vi "ControllerUI_New_Final.vi"() -> ()   [LabVIEW 2026]
uses:
  <vilib>/Utility/error.llb/Trim Whitespace One-Sided.vi
  <userlib>/_OpenG.lib/file/file.llb/openg_file.lvlib
panel:
  in  "Tab Control":T1(tab)
  out "background 2":picture
  in  "5-Day Rainstorm-to-Flood":bool
  out "script Status":string
  in  "voltage 1":dbl
  in  "DESD4 SOC":dbl(slide) step=1.0 scale=0.0..100.0 scale format="%#.6g"
  in  "DESD3 SOC":dbl(slide) step=1.0 scale=0.0..100.0 scale format="%#.6g"
  in  "DESD2 SOC":dbl(slide) step=1.0 scale=0.0..100.0 scale format="%#.6g"
  in  "wind speed":dbl(knob) caption="Wind Speed (m/s)" min=0.0 max=30.0 step=0.5 scale=0.0..255.0
  in  "stop":bool
  in  "Send UDP Command":bool caption="IO Building Send"
  out "Device Badge":string
  out "Selected Summary":string
  out "Device Description":string
  out "Device Name":string
  in  "DESD1 SOC":dbl(slide) step=1.0 scale=0.0..100.0 scale format="%#.6g"
  in  "BTN_DESD_4":bool
  in  "BTN_PV_1":bool
  in  "BTN_DESD_2":bool
  in  "BTN_Gen_1":bool
  in  "BTN_DESD_1":bool
  in  "BTN_Gen_2":bool
  in  "BTN_DESD_3":bool
  in  "BTN_PV_2":bool
  in  "BTN_Load_2":bool
  in  "BTN_Load_4":bool
  in  "BTN_Grid_1":bool
  in  "BTN_Load_3":bool
  in  "BTN_Wind_Turbine":bool
  out "background":picture
  in  "IO 1":bool
  in  "IO 2":bool
  in  "IO 3":bool
  in  "IO 4":bool
  in  "IO 6":bool
  in  "IO 7":bool
  in  "IO 8":bool
  in  "IO 5":bool
  in  "IO 9":bool
  in  "IO 10":bool
  in  "IO 11":bool
  in  "IO 12":bool
  in  "IO 13":bool
  in  "IO 14":bool
  in  "IO 15":bool
  in  "IO 16":bool
  in  "voltage 2":dbl
  in  "voltage 3":dbl
  in  "voltage 4":dbl
  # "LabVIEW-Based Physical Sandbox Intelligent Control System"
  # "LabVIEW-Based Physical Sandbox Intelligent Control System"
  # "Node Information"
  # "Control Panel"
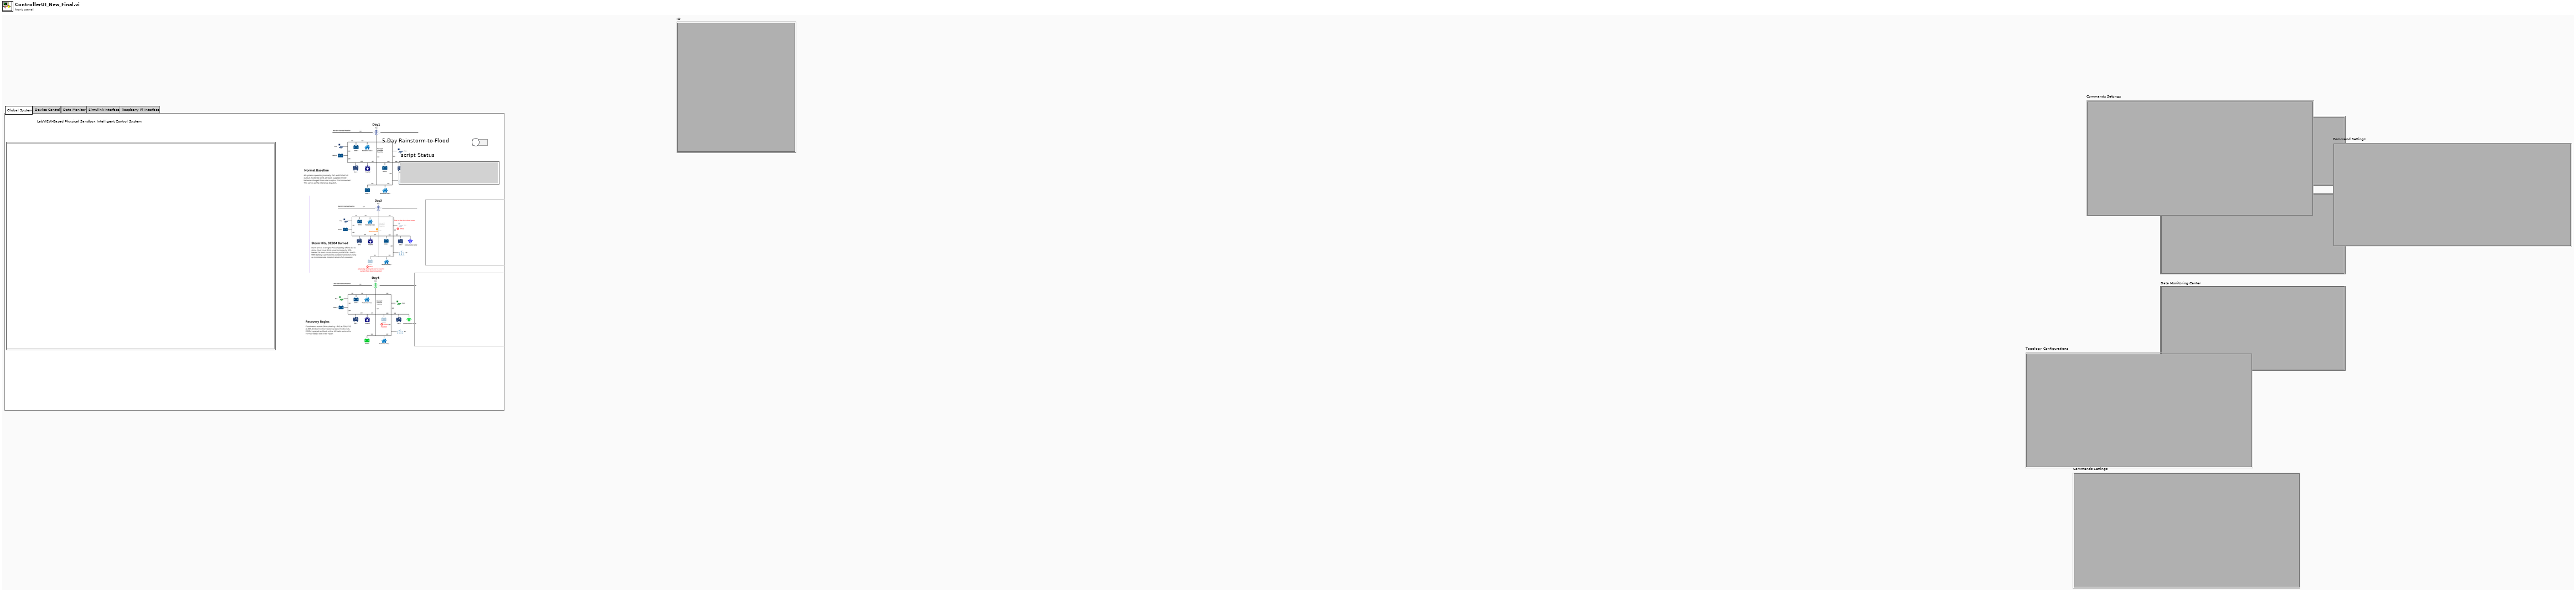
[diagram p1: front panel]
types:
  T1 = enum32{"Global System", "Device Control", "Data Monitor", "Simulink Interface", "Raspberry Pi Interface"}
  T2 = typedef "imagedata.ctl" = cluster{"image type":i32, "image depth":i32, "image":u8[], "mask":u8[], "colors":u32[], "Rectangle":cluster{"left":i16, "top":i16, "right":i16, "bottom":i16}}
  T3 = cluster{string, "wind speed":dbl, i32, i32, i32, i32}
  T4 = cluster{string, " DESD4 SOC":dbl, dbl, dbl, i32, i32}
  T5 = cluster{string, " DESD3 SOC":dbl, dbl, dbl, i32, i32}
  T6 = cluster{string, " DESD2 SOC":dbl, dbl, dbl, i32, i32}
  T7 = cluster{string, " DESD1 SOC":dbl, dbl, dbl, i32, i32}
  T8 = cluster{string, " DESD4 SOC":dbl, dbl, dbl, i32, i32}[]
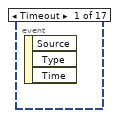
[diagram p2: hidden frame]
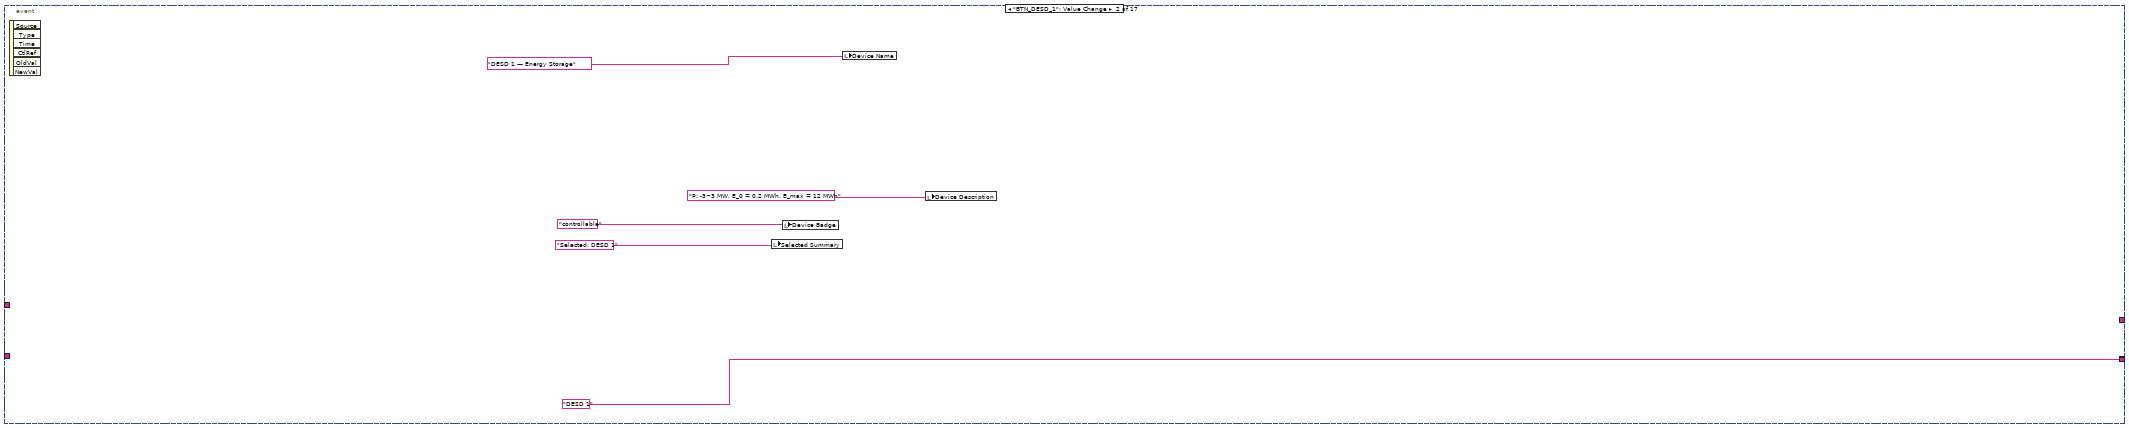
[diagram p3: hidden frame]
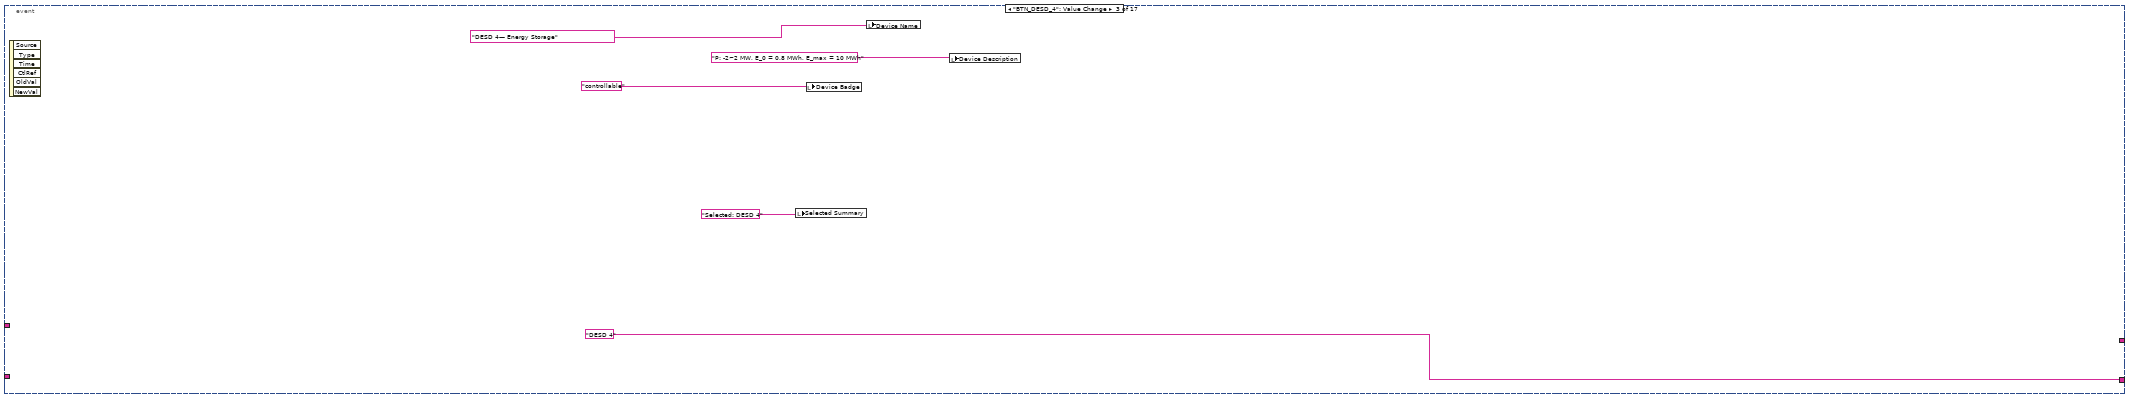
[diagram p4: hidden frame]
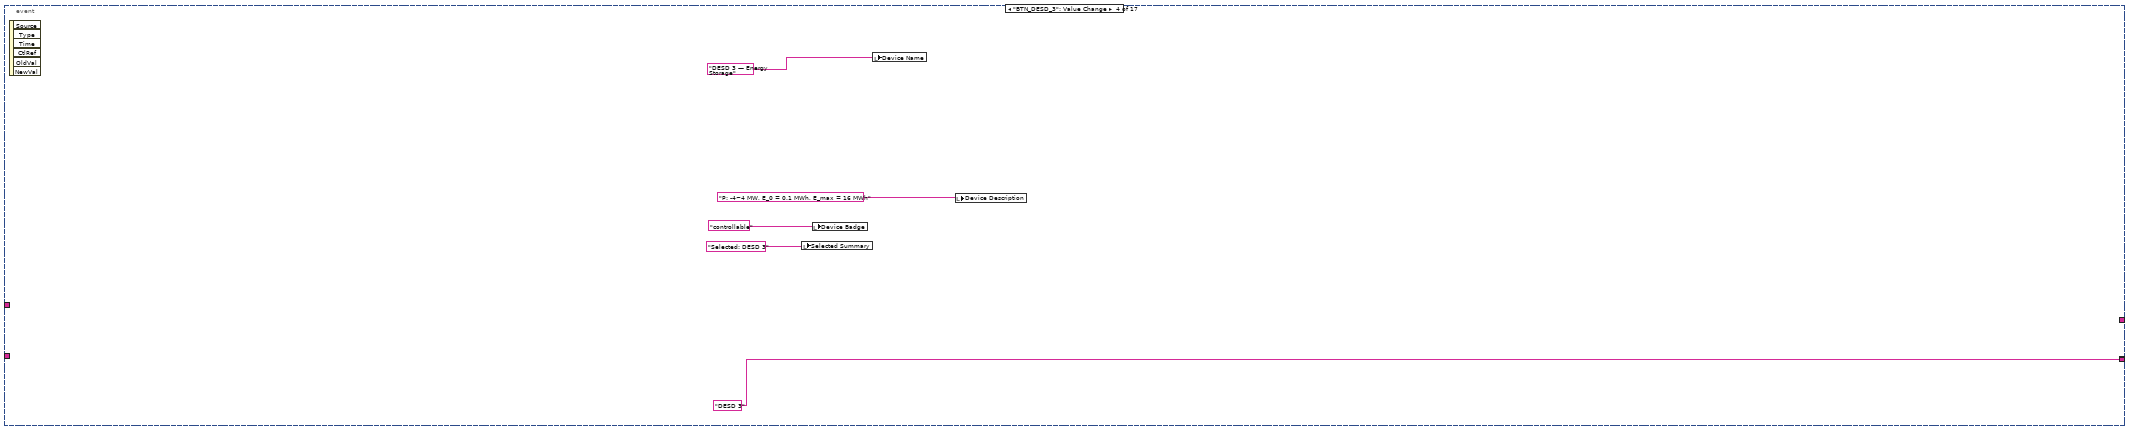
[diagram p5: hidden frame]
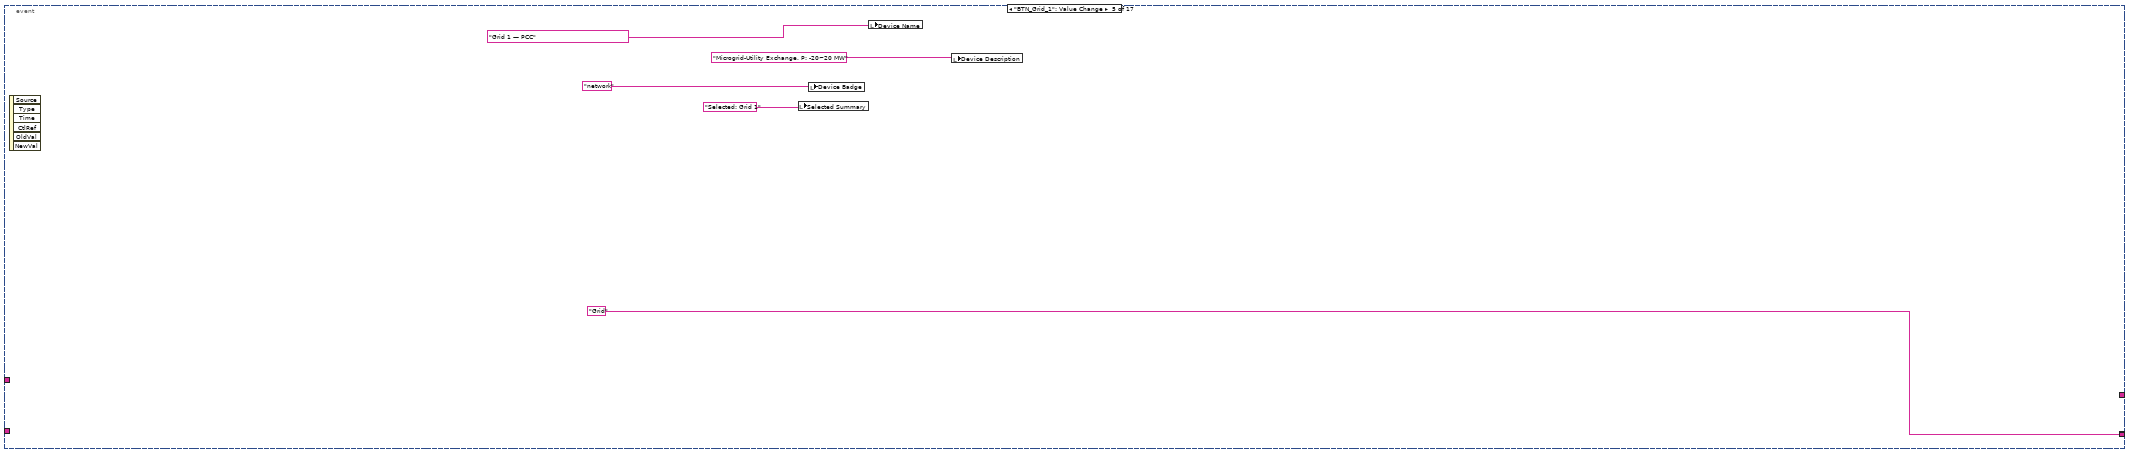
[diagram p6: hidden frame]
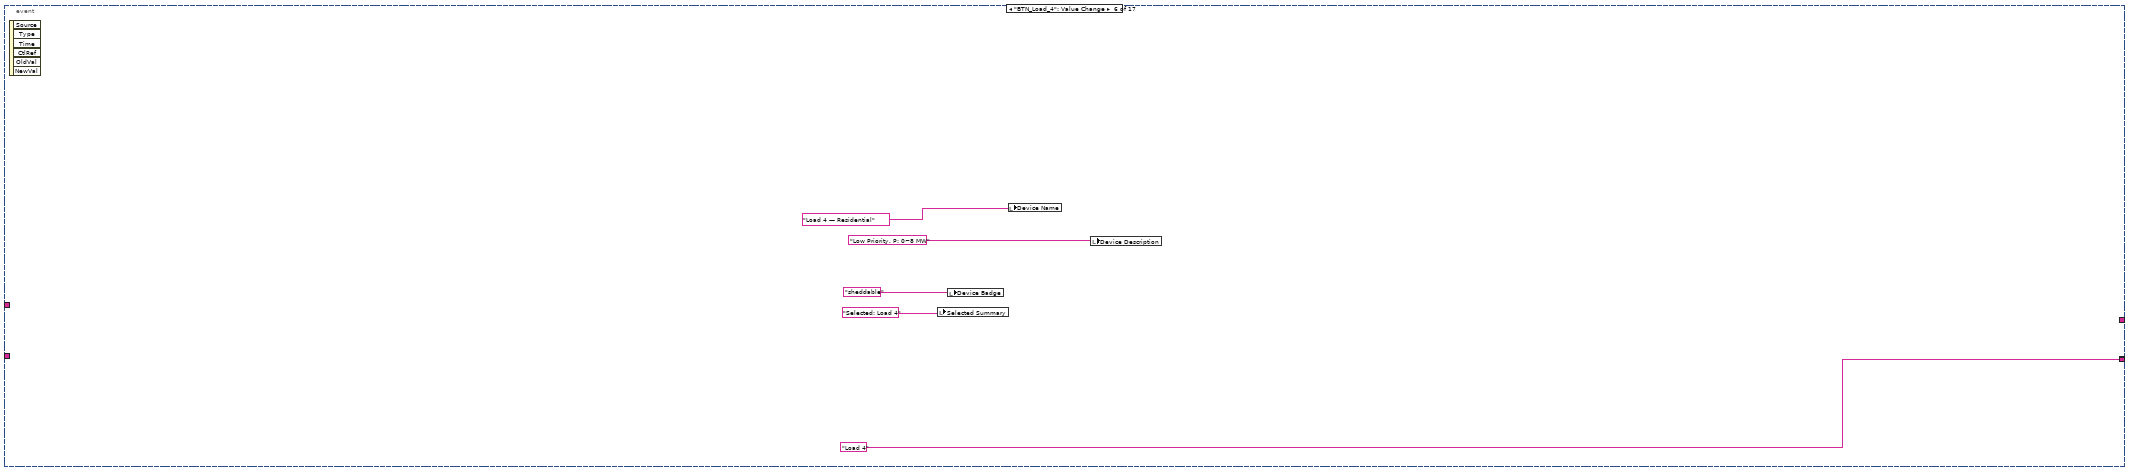
[diagram p7: hidden frame]
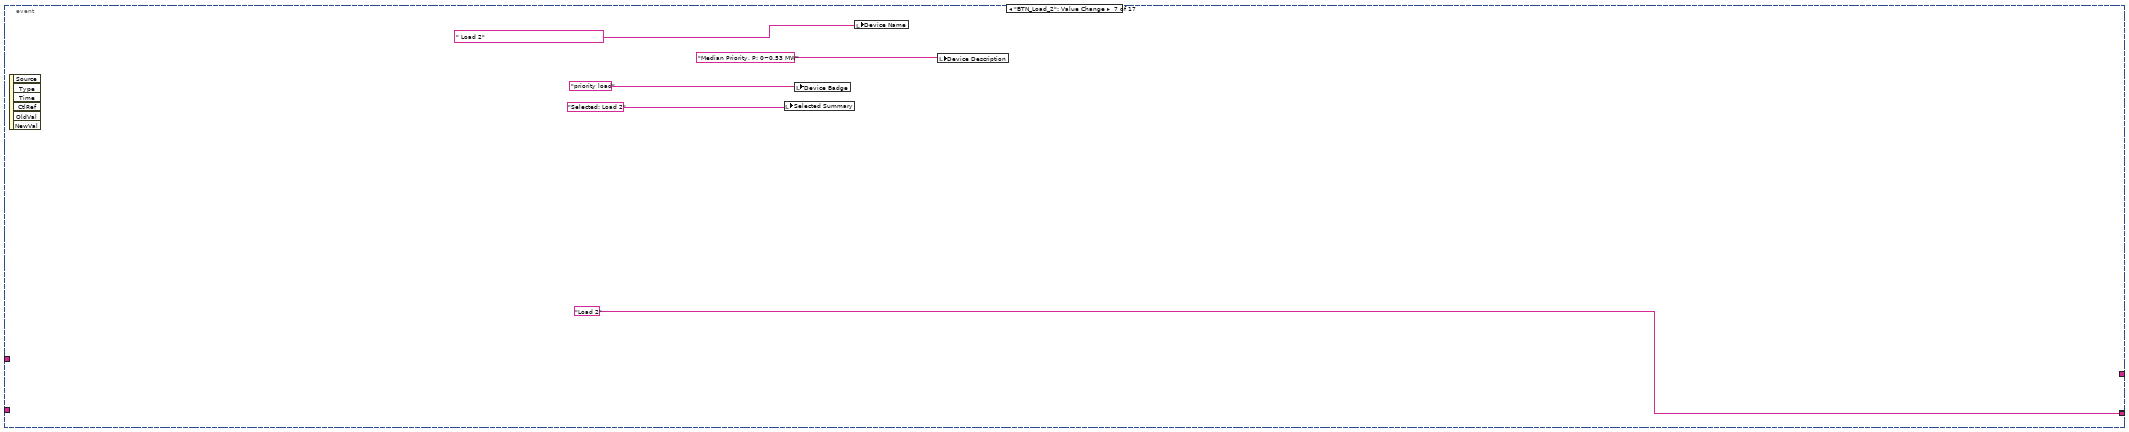
[diagram p8: hidden frame]
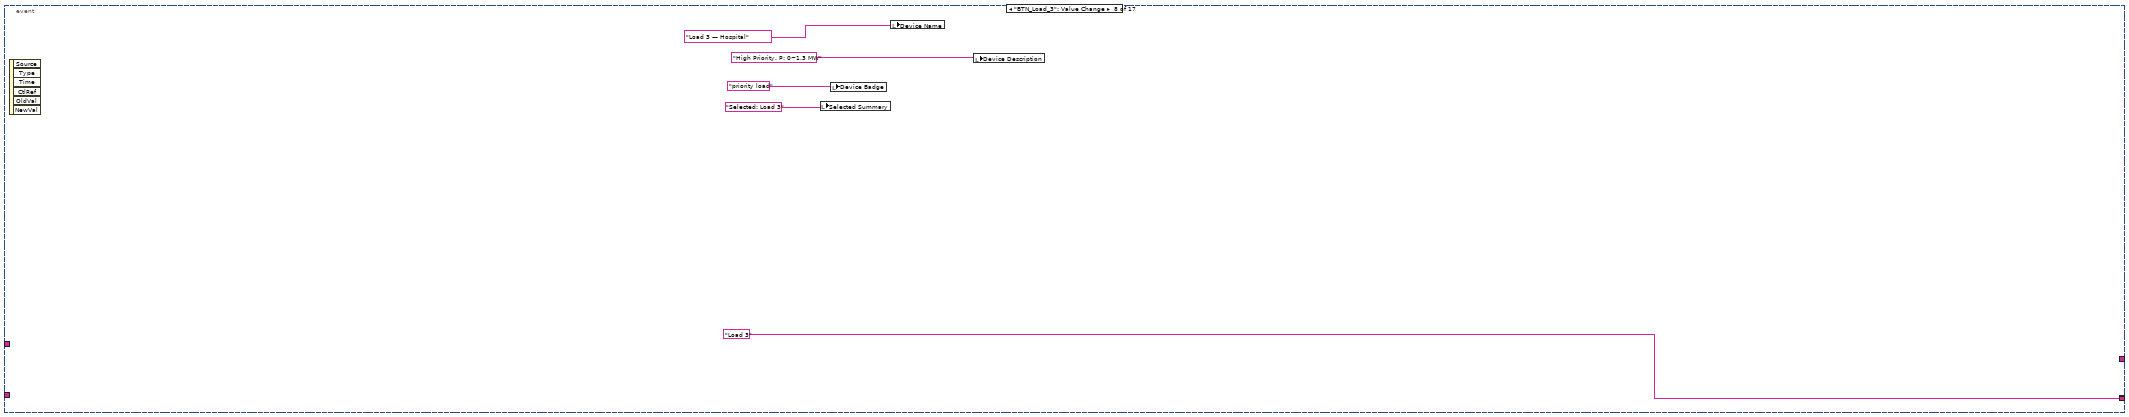
[diagram p9: hidden frame]
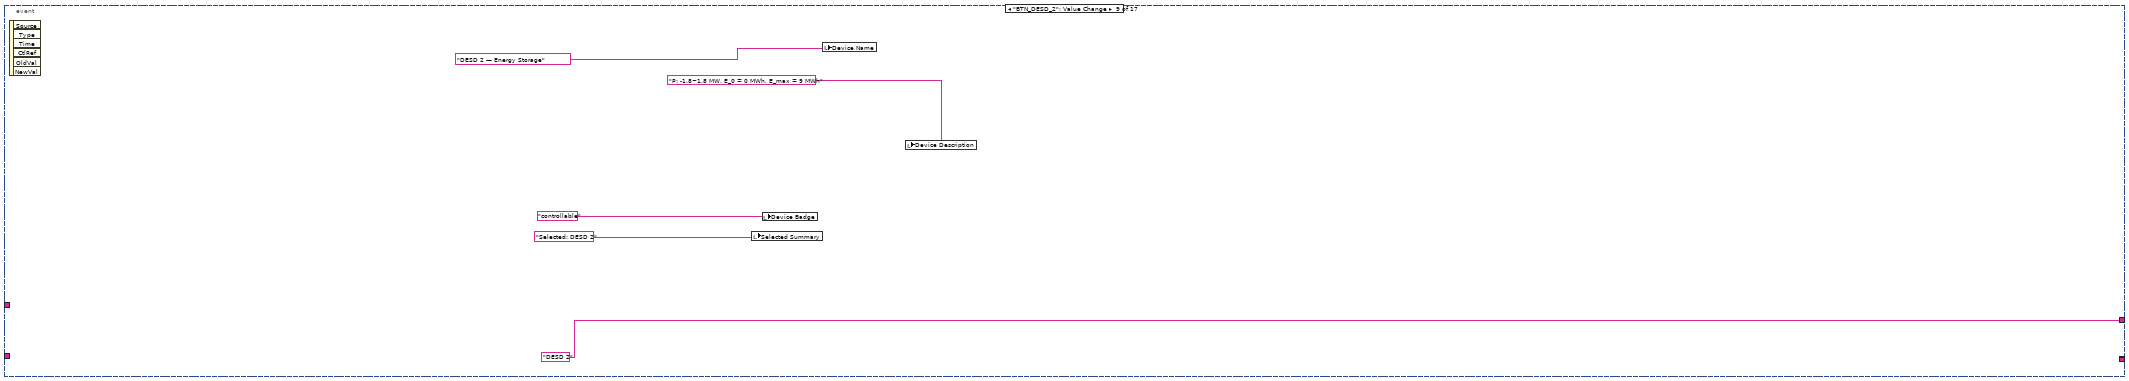
[diagram p10: hidden frame]
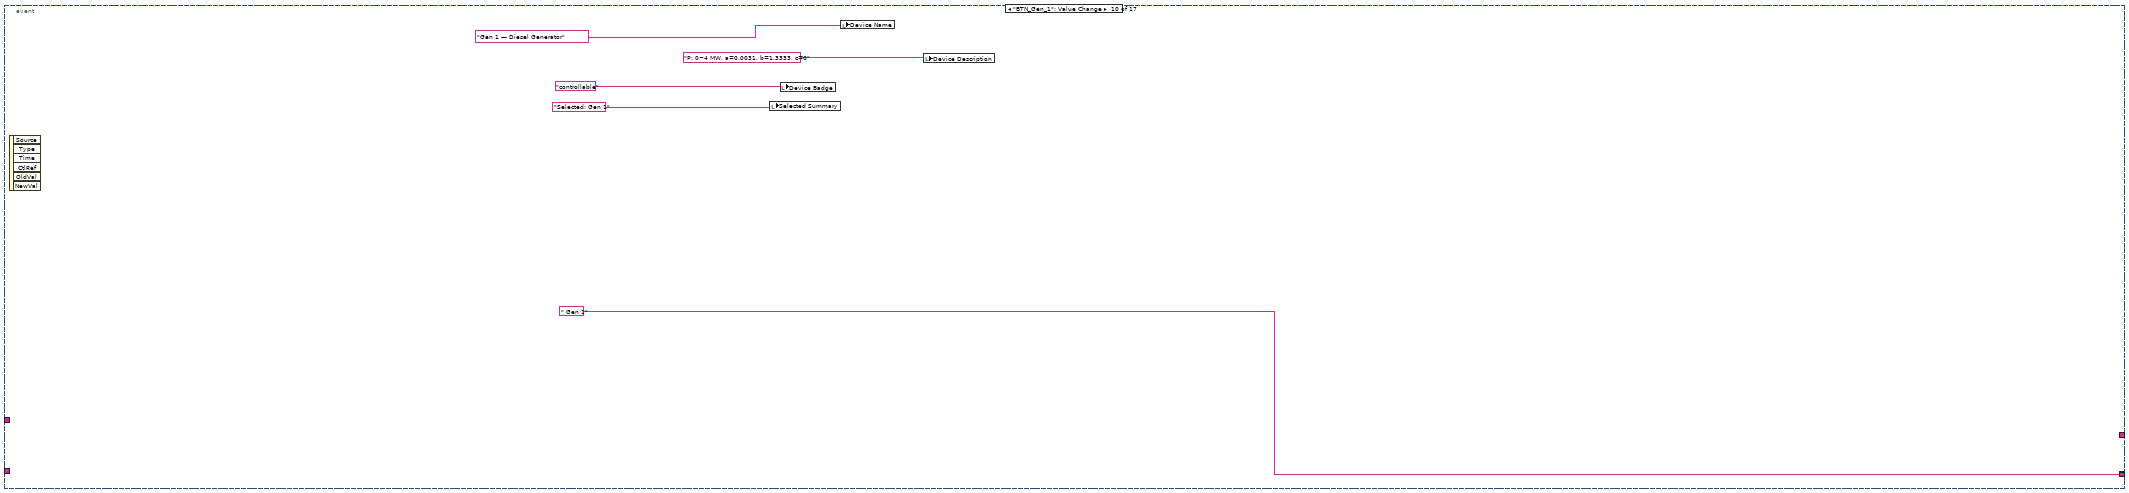
[diagram p11: hidden frame]
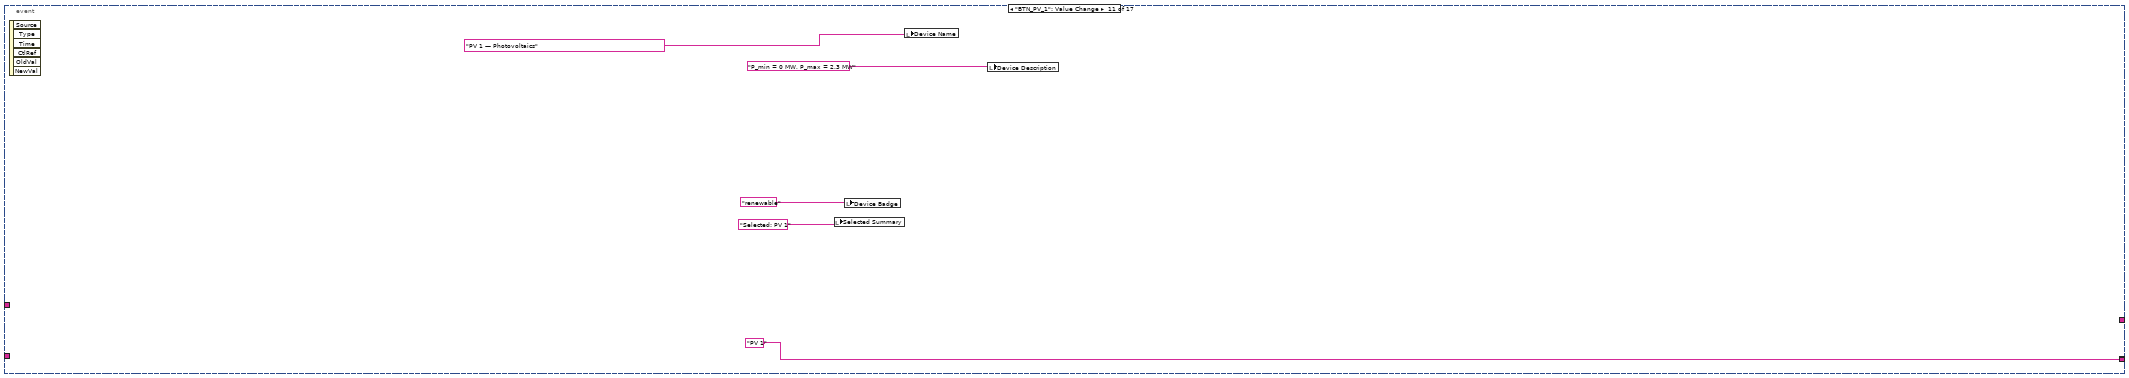
[diagram p12: hidden frame]
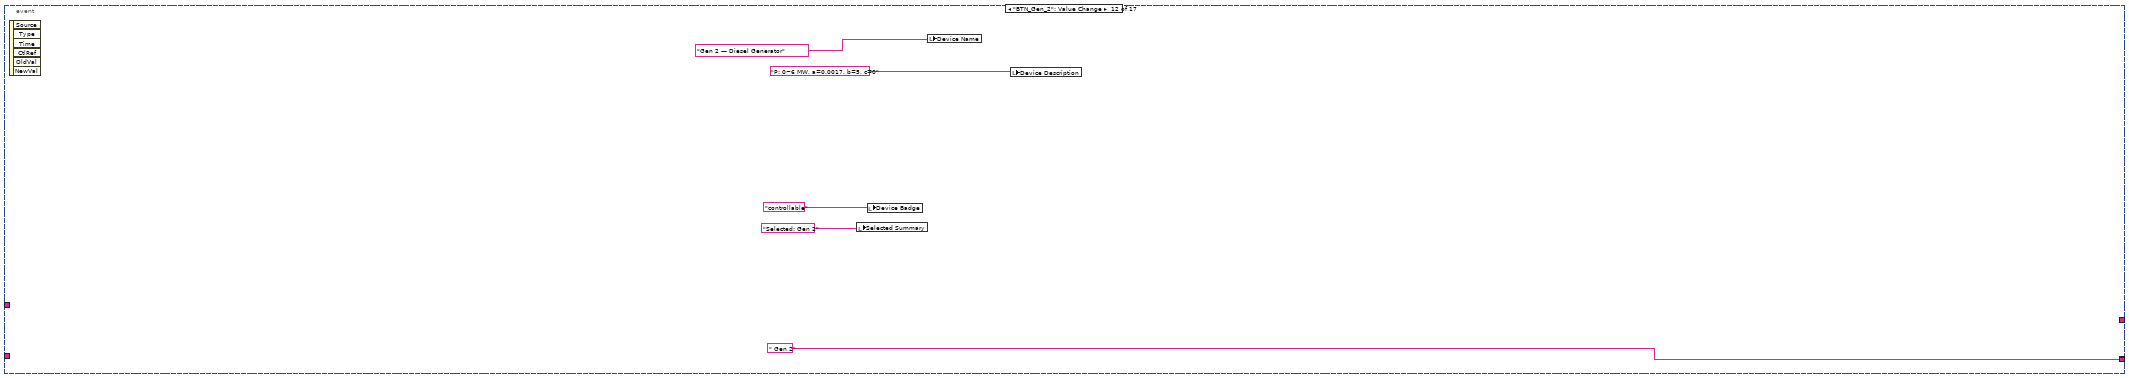
[diagram p13: hidden frame]
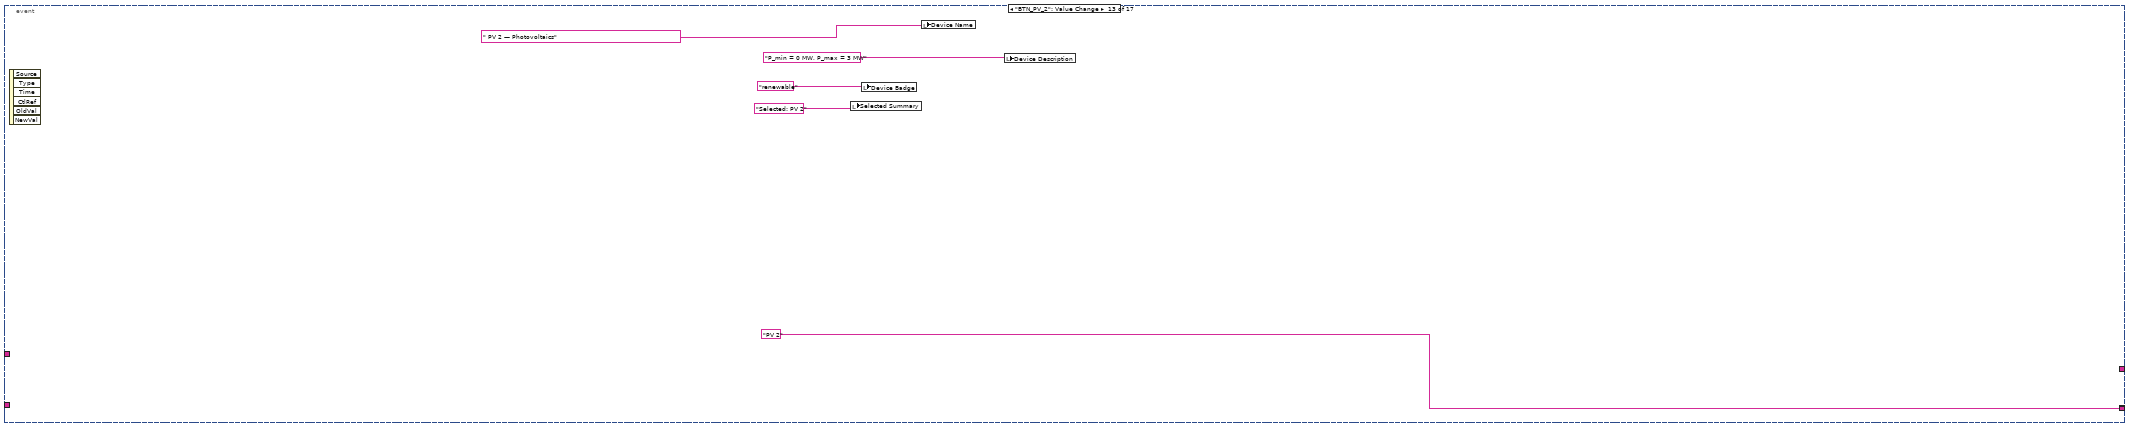
[diagram p14: hidden frame]
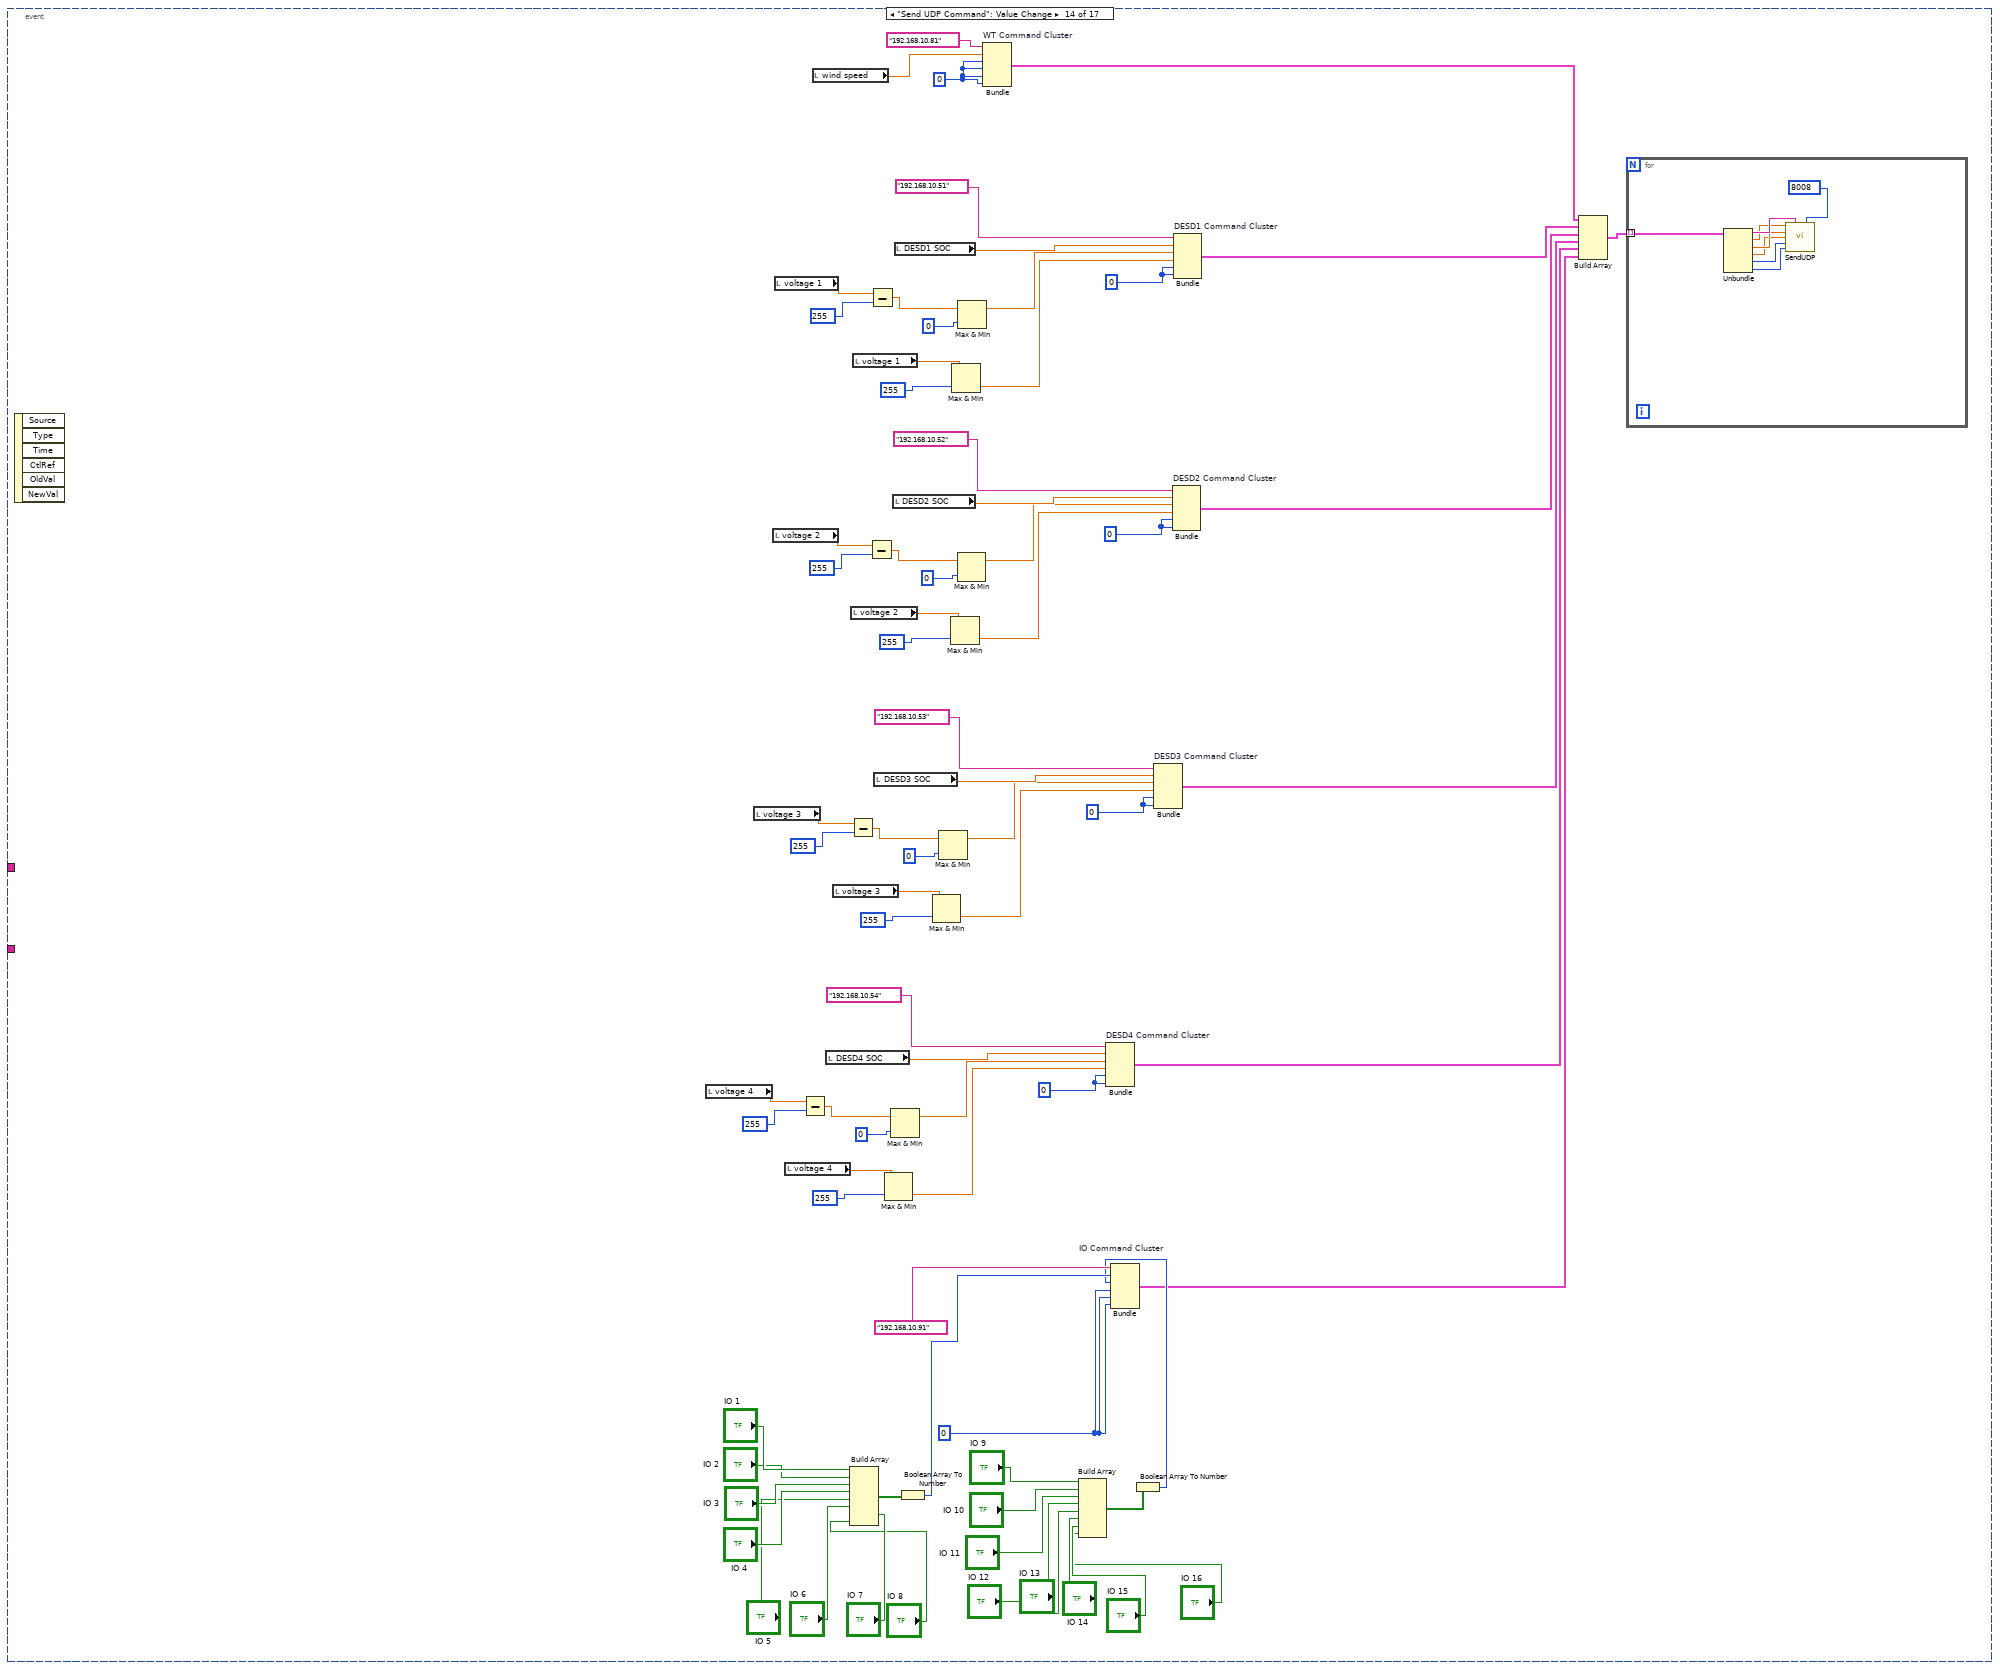
[diagram p15: hidden frame]
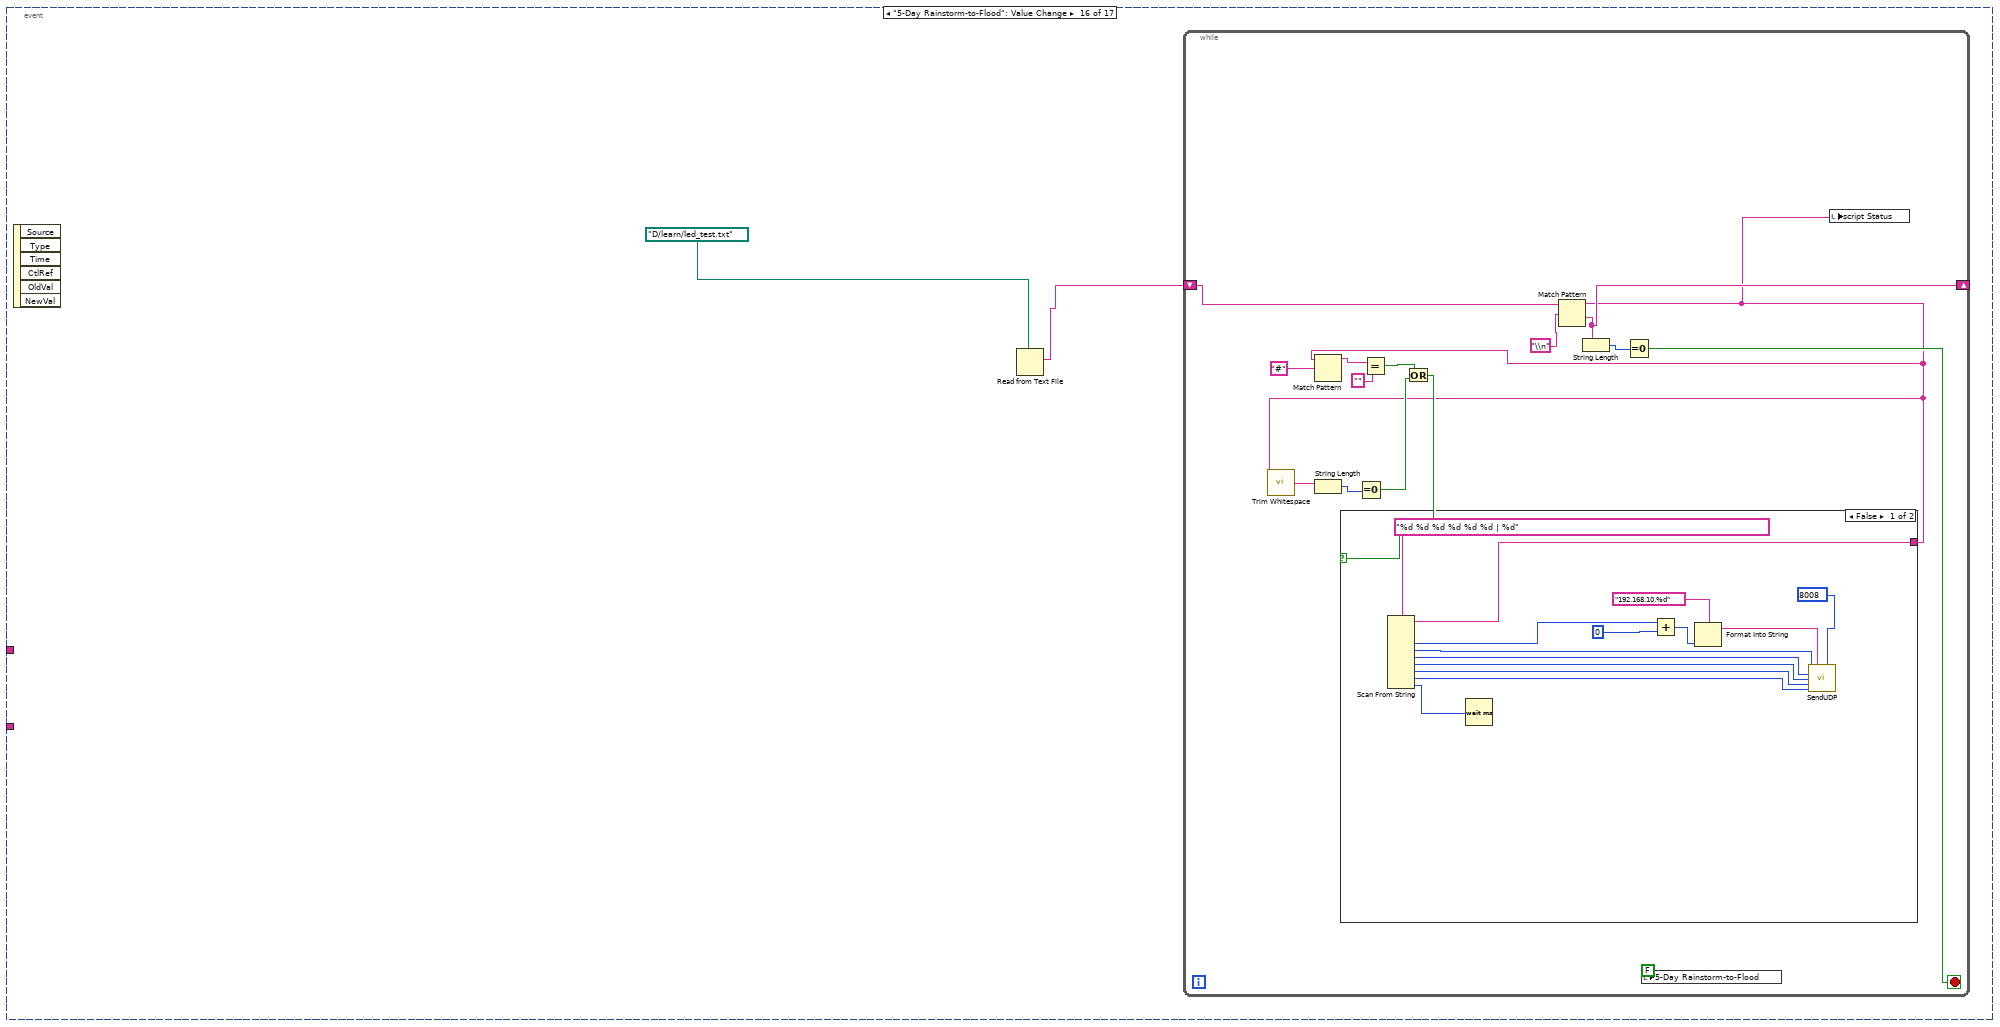
[diagram p16: hidden frame]
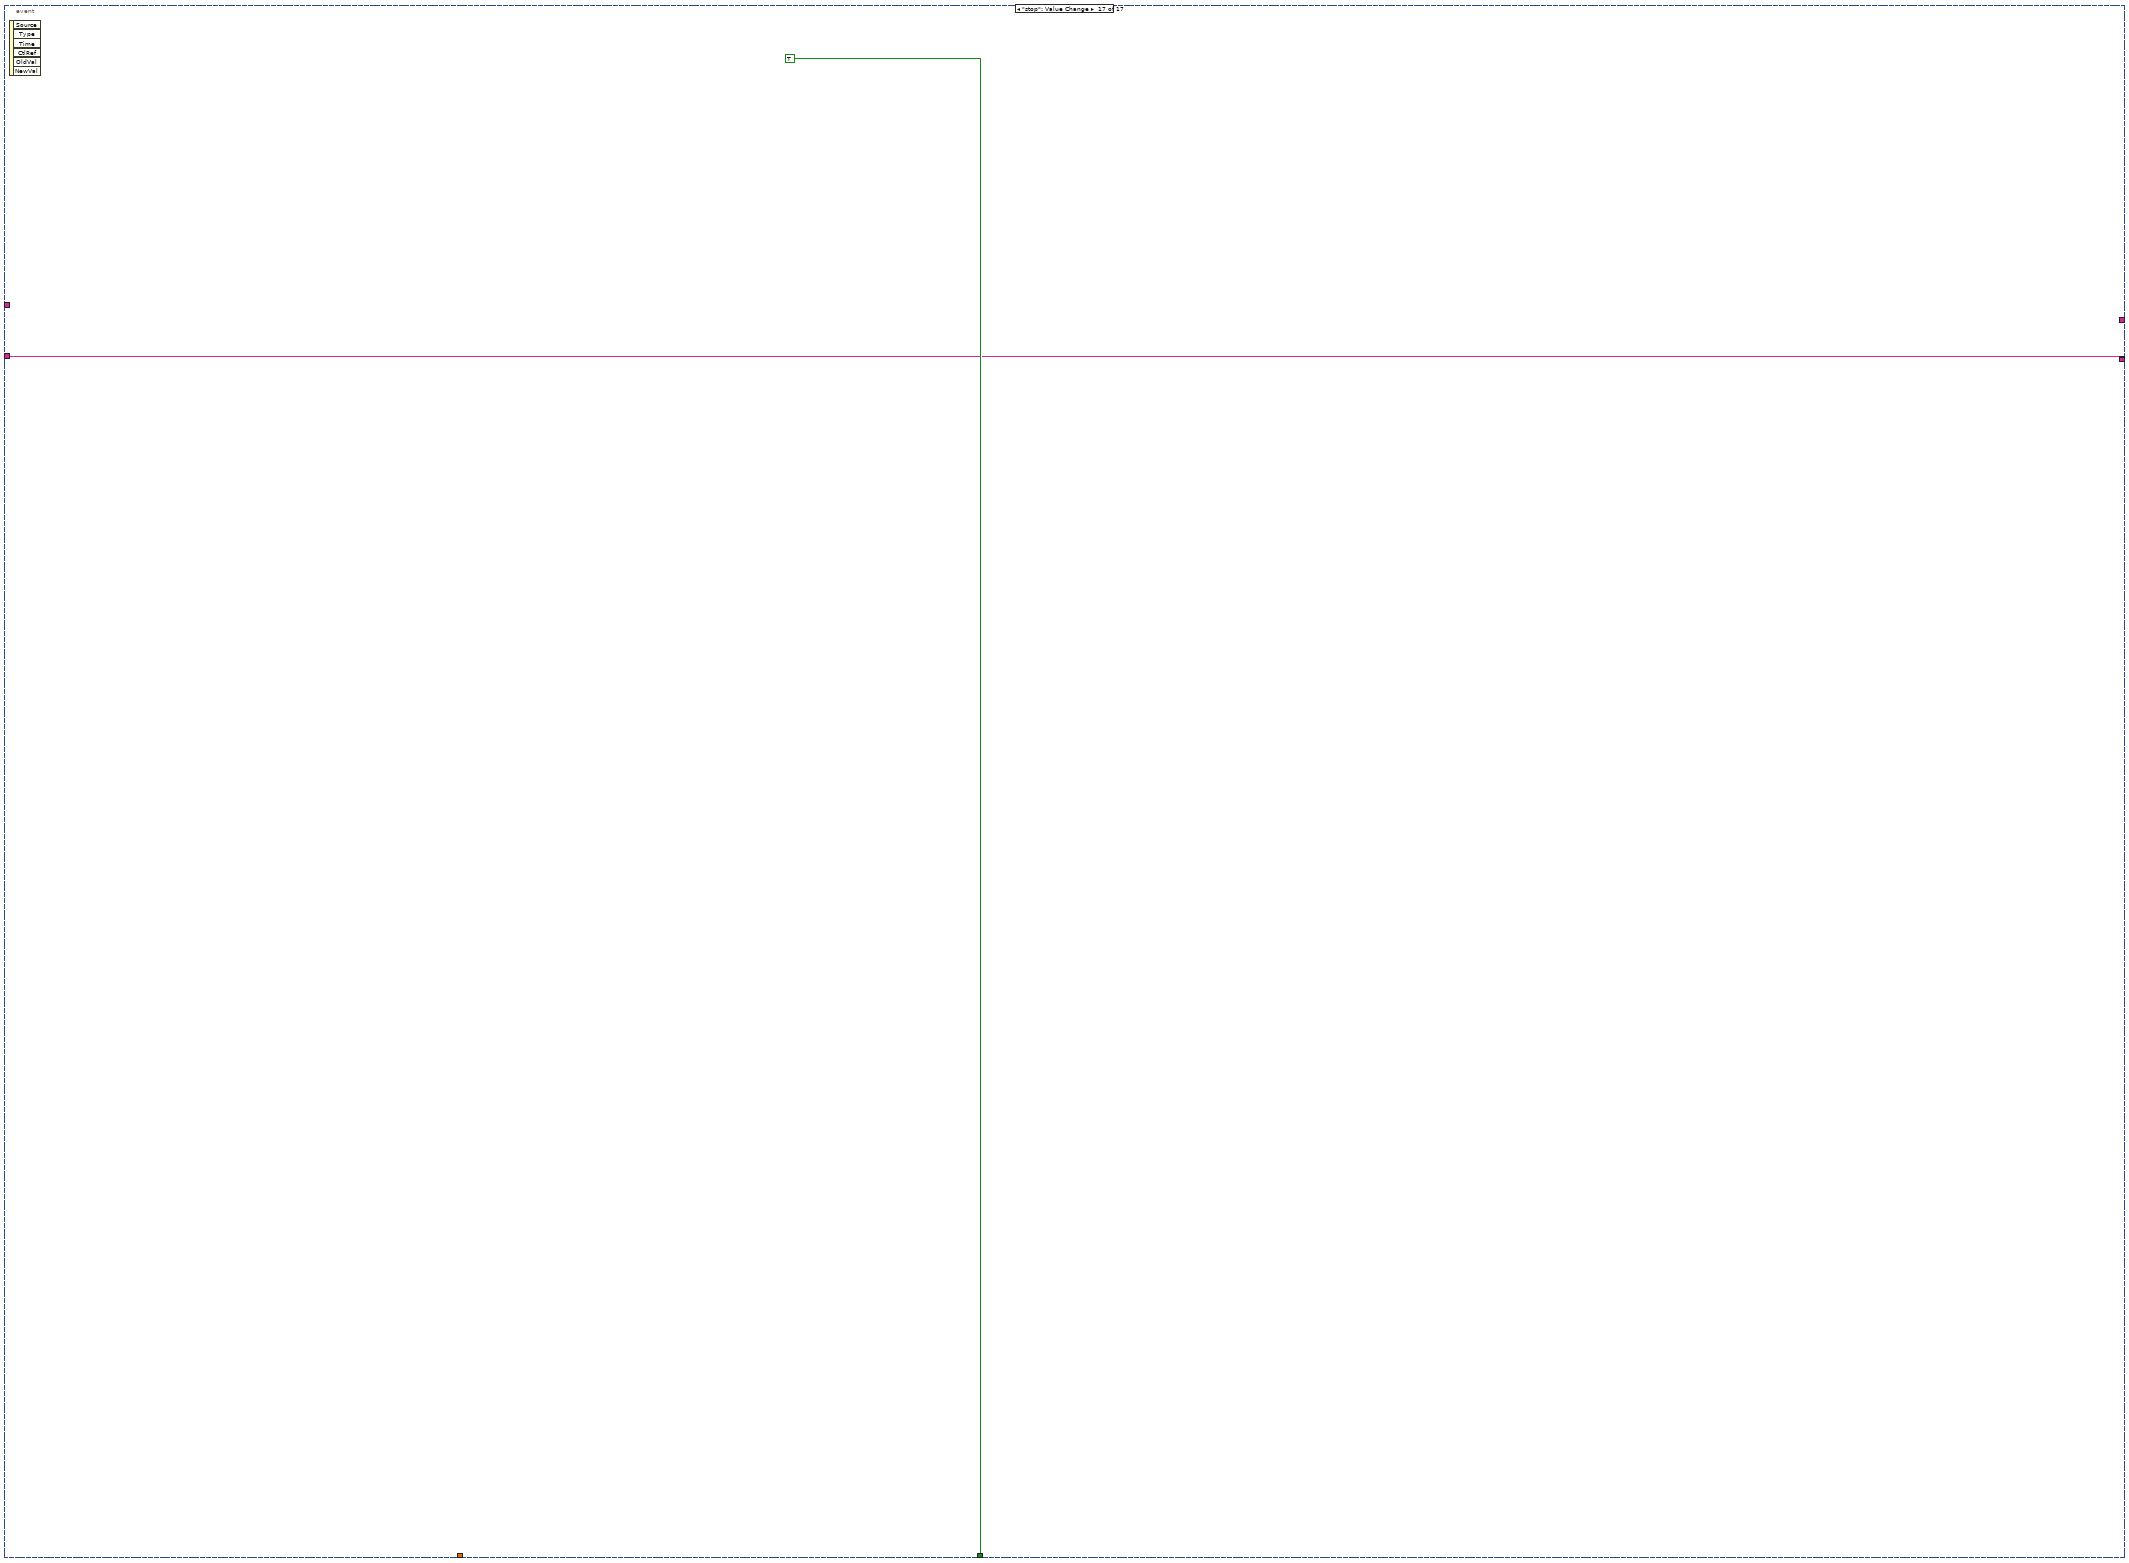
[diagram p18: hidden frame]
diagram:
  n1 = call <vilib>:"Read PNG File.vi"("path to PNG file"=path "ip-2D-final.png") -> ("image data"=w54:T2)  [unwired: 8 in, 2 out]
  n2 = property on="background" class="Pict"("ZoomFactor"=sgl 0.6 ("Zoom Factor")) -> ()  [unwired: 2 in, 2 out]
  n3 = call <vilib>:"Draw Flattened Pixmap.vi"("image data"=w54) -> ("new picture"=→"background":picture)  [unwired: 8 in]
  n4 = while {
    shift-right: [w56] -> _
    shift-left: "none" -> [w55]
    stop <- w58 stop-if-true
    n5 = event shown="[14] \"BTN_Wind_Turbine\": Value Change" {
      selector: _ -> [_ _ _ _ _ _ _ _ _ _ _ _ _ _ _ _ _]
      dyn-events: _ -> [_ _ _ _ _ _ _ _ _ _ _ _ _ _ _ _ _]
      timeout: _ -> [_ _ _ _ _ _ _ _ _ _ _ _ _ _ _ _ _]
      tunnel: [_ _ _ _ _ _ _ _ _ _ _ _ _ _ _ _ TRUE] -> w58
      tunnel: [_ _ _ _ _ _ _ _ "DESD 2" _ _ _ _ _ _ _ _] -> _
      tunnel: "wind speed" -> [_ _ _ _ _ _ _ _ _ _ _ _ _ _ _ _ _]
      tunnel: [_ "DESD 1" "DESD 4" "DESD 3" "Grid" "Load 4" "Load 2" "Load 3" _ " Gen 1" "PV 1" " Gen 2" _ _ "wind-turbine" _ w239] -> w56
      tunnel: w55 -> [_ _ _ _ _ _ _ _ _ _ _ _ _ _ _ _ _]
      tunnel: w55 -> [_ _ _ _ _ _ _ _ _ _ _ _ _ _ _ _ w239]
      tunnel: [_ _ _ _ _ _ _ _ _ _ _ _ "PV 2" _ _ _ _] -> _
      event Timeout {
        n6 = event-data() -> ()  [unwired: 1 in, 3 out]
      }
      event "BTN_DESD_1": Value Change {
        n7 = event-data() -> ()  [unwired: 1 in, 6 out]
        n8 = local write "Selected Summary"("Selected: DESD 1") -> ()
        n9 = local write "Device Badge"("controllable") -> ()
        n10 = local write "Device Name"("DESD 1 — Energy Storage") -> ()
        n11 = local write "Device Description"("P: -3~3 MW, E_0 = 0.2 MWh, E_max = 12 MWh") -> ()
      }
      event "BTN_DESD_4": Value Change {
        n12 = event-data() -> ()  [unwired: 1 in, 6 out]
        n13 = local write "Selected Summary"("Selected: DESD 4") -> ()
        n14 = local write "Device Badge"("controllable") -> ()
        n15 = local write "Device Name"("DESD 4— Energy Storage") -> ()
        n16 = local write "Device Description"("P: -2~2 MW, E_0 = 0.8 MWh, E_max = 10 MWh") -> ()
      }
      event "BTN_DESD_3": Value Change {
        n17 = event-data() -> ()  [unwired: 1 in, 6 out]
        n18 = local write "Selected Summary"("Selected: DESD 3") -> ()
        n19 = local write "Device Badge"("controllable") -> ()
        n20 = local write "Device Name"("DESD 3 — Energy Storage") -> ()
        n21 = local write "Device Description"("P: -4~4 MW, E_0 = 0.1 MWh, E_max = 16 MWh") -> ()
      }
      event "BTN_Grid_1": Value Change {
        n22 = event-data() -> ()  [unwired: 1 in, 6 out]
        n23 = local write "Selected Summary"("Selected: Grid 1") -> ()
        n24 = local write "Device Badge"("network") -> ()
        n25 = local write "Device Name"("Grid 1 — PCC") -> ()
        n26 = local write "Device Description"("Microgrid-Utility Exchange. P: -20~20 MW") -> ()
      }
      event "BTN_Load_4": Value Change {
        n27 = event-data() -> ()  [unwired: 1 in, 6 out]
        n28 = local write "Selected Summary"("Selected: Load 4") -> ()
        n29 = local write "Device Badge"("sheddable") -> ()
        n30 = local write "Device Name"("Load 4 — Residential") -> ()
        n31 = local write "Device Description"("Low Priority. P: 0~8 MW") -> ()
      }
      event "BTN_Load_2": Value Change {
        n32 = event-data() -> ()  [unwired: 1 in, 6 out]
        n33 = local write "Selected Summary"("Selected: Load 2") -> ()
        n34 = local write "Device Badge"("priority load") -> ()
        n35 = local write "Device Name"(" Load 2") -> ()
        n36 = local write "Device Description"("Median Priority. P: 0~0.53 MW") -> ()
      }
      event "BTN_Load_3": Value Change {
        n37 = event-data() -> ()  [unwired: 1 in, 6 out]
        n38 = local write "Selected Summary"("Selected: Load 3") -> ()
        n39 = local write "Device Badge"("priority load") -> ()
        n40 = local write "Device Name"("Load 3 — Hospital") -> ()
        n41 = local write "Device Description"("High Priority. P: 0~1.3 MW") -> ()
      }
      event "BTN_DESD_2": Value Change {
        n42 = event-data() -> ()  [unwired: 1 in, 6 out]
        n43 = local write "Selected Summary"("Selected: DESD 2") -> ()
        n44 = local write "Device Badge"("controllable") -> ()
        n45 = local write "Device Name"("DESD 2 — Energy Storage") -> ()
        n46 = local write "Device Description"("P: -1.8~1.8 MW, E_0 = 0 MWh, E_max = 9 MWh") -> ()
      }
      event "BTN_Gen_1": Value Change {
        n47 = event-data() -> ()  [unwired: 1 in, 6 out]
        n48 = local write "Selected Summary"("Selected: Gen 1") -> ()
        n49 = local write "Device Badge"("controllable") -> ()
        n50 = local write "Device Name"("Gen 1 — Diesel Generator") -> ()
        n51 = local write "Device Description"("P: 0~4 MW, a=0.0031, b=1.3333, c=0") -> ()
      }
      event "BTN_PV_1": Value Change {
        n52 = event-data() -> ()  [unwired: 1 in, 6 out]
        n53 = local write "Selected Summary"("Selected: PV 1") -> ()
        n54 = local write "Device Badge"("renewable") -> ()
        n55 = local write "Device Name"("PV 1 — Photovoltaics") -> ()
        n56 = local write "Device Description"("P_min = 0 MW, P_max = 2.3 MW") -> ()
      }
      event "BTN_Gen_2": Value Change {
        n57 = event-data() -> ()  [unwired: 1 in, 6 out]
        n58 = local write "Selected Summary"("Selected: Gen 2") -> ()
        n59 = local write "Device Badge"("controllable") -> ()
        n60 = local write "Device Name"("Gen 2 — Diesel Generator") -> ()
        n61 = local write "Device Description"("P: 0~6 MW, a=0.0017, b=5, c=0") -> ()
      }
      event "BTN_PV_2": Value Change {
        n62 = event-data() -> ()  [unwired: 1 in, 6 out]
        n63 = local write "Selected Summary"("Selected: PV 2") -> ()
        n64 = local write "Device Badge"("renewable") -> ()
        n65 = local write "Device Name"(" PV 2 — Photovoltaics") -> ()
        n66 = local write "Device Description"("P_min = 0 MW, P_max = 3 MW") -> ()
      }
      event "Send UDP Command": Value Change {
        w130 = 0
        w141 = 0
        w152 = 0
        w163 = 0
        w175 = 0
        w126 = 0
        n67 = event-data() -> ()  [unwired: 1 in, 6 out]
        n68 = local read "voltage 4"() -> (w137:dbl)
        n69 = local read "voltage 3"() -> (w148:dbl)
        n70 = local read "voltage 2"() -> (w159:dbl)
        n71 = local read "voltage 1"() -> (w170:dbl)
        n72 = local read "voltage 4"() -> (w140:dbl)
        n73 = Subtract(x=w137, y=255) -> (x-y=w135:dbl)
        n74 = local read "wind speed"() -> (w174:dbl)
        n75 = local read "DESD4 SOC"() -> (w133:dbl)
        n76 = local read "voltage 3"() -> (w151:dbl)
        n77 = Subtract(x=w148, y=255) -> (x-y=w146:dbl)
        n78 = Build Array("IO 1", "IO 2", "IO 3", "IO 4", "IO 5", "IO 6", "IO 7", "IO 8") -> (w178:bool[])
        n79 = local read "voltage 2"() -> (w162:dbl)
        n80 = local read "voltage 1"() -> (w173:dbl)
        n81 = Subtract(x=w159, y=255) -> (x-y=w157:dbl)
        n82 = Subtract(x=w170, y=255) -> (x-y=w168:dbl)
        n83 = local read "DESD3 SOC"() -> (w144:dbl)
        n84 = Max & Min(x=w140, y=255) -> (min(x,y)=w131:dbl)  [unwired: 1 out]
        n85 = Max & Min(x=w135, y=0) -> (max(x,y)=w132:dbl)  [unwired: 1 out]
        n86 = local read "DESD2 SOC"() -> (w155:dbl)
        n87 = local read "DESD1 SOC"() -> (w166:dbl)
        n88 = Boolean Array To Number(Boolean array=w178) -> (number=w128:u32)
        n89 = Max & Min(x=w151, y=255) -> (min(x,y)=w142:dbl)  [unwired: 1 out]
        n90 = Max & Min(x=w146, y=0) -> (max(x,y)=w143:dbl)  [unwired: 1 out]
        n91 = Max & Min(x=w162, y=255) -> (min(x,y)=w153:dbl)  [unwired: 1 out]
        n92 = Max & Min(x=w173, y=255) -> (min(x,y)=w164:dbl)  [unwired: 1 out]
        n93 = Max & Min(x=w157, y=0) -> (max(x,y)=w154:dbl)  [unwired: 1 out]
        n94 = Max & Min(x=w168, y=0) -> (max(x,y)=w165:dbl)  [unwired: 1 out]
        n95 = Bundle "WT Command Cluster"("192.168.10.81", "wind speed"=w174, w175, w175, w175, w175) -> (w125:T3)  [unwired: 1 in]
        n96 = Build Array("IO 9", "IO 10", "IO 11", "IO 12", "IO 13", "IO 14", "IO 15", "IO 16") -> (w179:bool[])
        n97 = Bundle "DESD4 Command Cluster"("192.168.10.54", "DESD4 SOC"=w133, w132, w131, w130, w130) -> (w121:T4)  [unwired: 1 in]
        n98 = Boolean Array To Number(Boolean array=w179) -> (number=w127:u32)
        n99 = Bundle "IO Command Cluster"("192.168.10.91", w128, w127, w126, w126, w126) -> (w120:cluster{string, u32, u32, i32, i32, i32})  [unwired: 1 in]
        n100 = Bundle "DESD3 Command Cluster"("192.168.10.53", "DESD3 SOC"=w144, w143, w142, w141, w141) -> (w122:T5)  [unwired: 1 in]
        n101 = Bundle "DESD2 Command Cluster"("192.168.10.52", "DESD2 SOC"=w155, w154, w153, w152, w152) -> (w123:T6)  [unwired: 1 in]
        n102 = Bundle "DESD1 Command Cluster"("192.168.10.51", "DESD1 SOC"=w166, w165, w164, w163, w163) -> (w124:T7)  [unwired: 1 in]
        n103 = Build Array(w125, w124, w123, w122, w121, w120) -> (w119:T8)
        n104 = for {
          tunnel: w119 -> [w202] mode=indexing
          n105 = Unbundle(w202) -> (w201:string, "DESD4 SOC"=w200:dbl, w199:dbl, w198:dbl, w197:i32, w196:i32)
          n106 = call "SendUDP.vi"("Arg3"=w200, "IP"=w201, "Port"=8008, "Arg4"=w199, "Arg5"=w198, "Arg6"=w197, "Arg7"=w196) -> ()  [unwired: 9 in]
        }
      }
      event "BTN_Wind_Turbine": Value Change {
        n107 = event-data() -> ()  [unwired: 1 in, 6 out]
        n108 = local write "Device Name"("WT 1 — Wind Turbine") -> ()
        n109 = local write "Device Badge"("weather input") -> ()
        n110 = local write "Selected Summary"("Selected: WT 1") -> ()
        n111 = local write "Device Description"("P_min = 0 MW, P_max = 1.05 MW") -> ()
      }
      event "5-Day Rainstorm-to-Flood": Value Change {
        n112 = event-data() -> ()  [unwired: 1 in, 6 out]
        n113 = Read from Text File(file (use dialog)=path "D:/learn/led_test.txt") -> (text=w208:string)  [unwired: 3 in, 3 out]
        n114 = while {
          shift-right: [w213] -> _
          shift-left: w208 -> [w214]
          stop <- w212 stop-if-true
          n115 = Match Pattern(string=w214, regular expression="\\n") -> (before substring=w211:string, after substring=w213:string)  [unwired: 1 in, 2 out]
          n116 = call <vilib>:"Trim Whitespace.vi"("string"=w211) -> ("trimmed string"=w219:string)  [unwired: 1 in]
          n117 = Match Pattern(string=w211, regular expression="#") -> (before substring=w221:string)  [unwired: 1 in, 3 out]
          n118 = String Length(string=w219) -> (length=w218:i32)
          n119 = Equal To 0?(x=w218) -> (x = 0?=w216:bool)
          n120 = Equal?(x=w221, y="" ("regular expression")) -> (x = y?=w217:bool)
          n121 = Or(x=w217, y=w216) -> (x .or. y?=w215:bool)
          n122 = case shown="False" w215 {
            tunnel: w211 -> [w238 _]
            frame False {
              n123 = Scan From String(format string="%d %d %d %d %d %d | %d" ("regular expression"), input string=w238) -> (output 1=w236:i32, output 2=w230:u8, output 3=w229:u8, output 4=w228:u8, output 5=w227:u8, output 6=w226:u8, output 7=w225:i32)  [unwired: 9 in, 3 out]
              n124 = Wait (ms)(milliseconds to wait=w225) -> ()  [unwired: 1 out]
              n125 = Add(x=w236, y=0) -> (x+y=w235:i32)
              n126 = Format Into String(format string="192.168.10.%d", w235) -> (resulting string=w233:string)  [unwired: 2 in, 1 out]
              n127 = call "SendUDP.vi"("Arg3"=w230, "IP"=w233, "Port"=8008, "Arg4"=w229, "Arg5"=w228, "Arg6"=w227, "Arg7"=w226) -> ()  [unwired: 9 in]
            }
            frame True {
            }
          }
          n128 = String Length(string=w213) -> (length=w223:i32)
          n129 = Equal To 0?(x=w223) -> (x = 0?=w212:bool)
          n130 = local write "5-Day Rainstorm-to-Flood"(FALSE) -> ()
          n131 = local write "script Status"(w211) -> ()
        }
      }
      event "stop": Value Change {
        n132 = event-data() -> ()  [unwired: 1 in, 6 out]
      }
    }
  }
  n133 = call <userlib>:"Current VI's Path__ogtk.vi"() -> ("Current VI's Path (+ Relative)"=w41:path)  [unwired: 1 in]
  n134 = call <userlib>:"Current VI's Path__ogtk.vi"() -> ("Current VI's Path (+ Relative)"=w47:path)  [unwired: 1 in]
  n135 = control-ref of="Command Settings"() -> (w30:refnum<vi>)
  n136 = Strip Path(path=w41) -> (stripped path=w40:path)  [unwired: 1 out]
  n137 = Strip Path(path=w47) -> (stripped path=w46:path)  [unwired: 1 out]
  n138 = control-ref of="Scenario Parameters Settings"() -> (w31:refnum<vi>)
  n139 = control-ref of="Timeline Configurations"() -> (w8:refnum<vi>)
  n140 = Build Path(base path=w40, name or relative path="raspberry_pi_control_panel.vi") -> (appended path=w38:path)
  n141 = Build Path(base path=w46, name or relative path="system_config.vi") -> (appended path=w44:path)
  n142 = Open VI Reference(vi path=w38) -> (vi reference=w43:refnum<vi>)  [unwired: 5 in, 1 out]
  n143 = Open VI Reference(vi path=w44) -> (vi reference=w49:refnum<vi>)  [unwired: 5 in, 1 out]
  n144 = invoke class="SubPnl" method="Insert VI"(reference=w30, "VI Ref"=w43) -> ()  [unwired: 2 in, 4 out]
  n145 = invoke class="SubPnl" method="Insert VI"(reference=w31, "VI Ref"=w49) -> ()  [unwired: 2 in, 4 out]
  n146 = call <userlib>:"Current VI's Path__ogtk.vi"() -> ("Current VI's Path (+ Relative)"=w12:path)  [unwired: 1 in]
  n147 = invoke class="VI" method="Run VI"(reference=w43, "Wait until done"=FALSE ("Wait Until Done")) -> ()  [unwired: 3 in, 5 out]
  n148 = invoke class="VI" method="Run VI"(reference=w49, "Wait until done"=FALSE ("Wait Until Done")) -> ()  [unwired: 3 in, 5 out]
  n149 = Strip Path(path=w12) -> (stripped path=w11:path)  [unwired: 1 out]
  n150 = control-ref of="Data Monitoring"() -> (w29:refnum<vi>)
  n151 = Build Path(base path=w11, name or relative path="timeline_config.vi") -> (appended path=w9:path)
  n152 = Open VI Reference(vi path=w9) -> (vi reference=w14:refnum<vi>)  [unwired: 5 in, 1 out]
  n153 = call <userlib>:"Current VI's Path__ogtk.vi"() -> ("Current VI's Path (+ Relative)"=w35:path)  [unwired: 1 in]
  n154 = invoke class="SubPnl" method="Insert VI"(reference=w8, "VI Ref"=w14) -> ()  [unwired: 2 in, 4 out]
  n155 = Strip Path(path=w35) -> (stripped path=w34:path)  [unwired: 1 out]
  n156 = invoke class="VI" method="Run VI"(reference=w14, "Wait until done"=FALSE ("Wait Until Done")) -> ()  [unwired: 3 in, 5 out]
  n157 = Build Path(base path=w34, name or relative path="monitoring_center.vi") -> (appended path=w32:path)
  n158 = Open VI Reference(vi path=w32) -> (vi reference=w37:refnum<vi>)  [unwired: 5 in, 1 out]
  n159 = invoke class="SubPnl" method="Insert VI"(reference=w29, "VI Ref"=w37) -> ()  [unwired: 2 in, 4 out]
  n160 = invoke class="VI" method="Run VI"(reference=w37, "Wait until done"=FALSE ("Wait Until Done")) -> ()  [unwired: 3 in, 5 out]
  n161 = control-ref of="Topology Configurations"() -> (w15:refnum<vi>)
  n162 = control-ref of="Commands Settings"() -> (w22:refnum<vi>)
  n163 = control-ref of="Simulink Data"() -> (w1:refnum<vi>)
  n164 = call <userlib>:"Current VI's Path__ogtk.vi"() -> ("Current VI's Path (+ Relative)"=w26:path)  [unwired: 1 in]
  n165 = call <userlib>:"Current VI's Path__ogtk.vi"() -> ("Current VI's Path (+ Relative)"=w19:path)  [unwired: 1 in]
  n166 = call <userlib>:"Current VI's Path__ogtk.vi"() -> ("Current VI's Path (+ Relative)"=w5:path)  [unwired: 1 in]
  n167 = Strip Path(path=w26) -> (stripped path=w25:path)  [unwired: 1 out]
  n168 = Strip Path(path=w19) -> (stripped path=w18:path)  [unwired: 1 out]
  n169 = Strip Path(path=w5) -> (stripped path=w4:path)  [unwired: 1 out]
  n170 = Build Path(base path=w25, name or relative path="translation_control_panel.vi") -> (appended path=w23:path)
  n171 = Open VI Reference(vi path=w23) -> (vi reference=w28:refnum<vi>)  [unwired: 5 in, 1 out]
  n172 = Build Path(base path=w18, name or relative path="topology_config.vi") -> (appended path=w16:path)
  n173 = Open VI Reference(vi path=w16) -> (vi reference=w21:refnum<vi>)  [unwired: 5 in, 1 out]
  n174 = invoke class="SubPnl" method="Insert VI"(reference=w22, "VI Ref"=w28) -> ()  [unwired: 2 in, 4 out]
  n175 = Build Path(base path=w4, name or relative path="GlobalMenuStatusStorage2.vi") -> (appended path=w2:path)
  n176 = Open VI Reference(vi path=w2) -> (vi reference=w7:refnum<vi>)  [unwired: 5 in, 1 out]
  n177 = invoke class="SubPnl" method="Insert VI"(reference=w15, "VI Ref"=w21) -> ()  [unwired: 2 in, 4 out]
  n178 = invoke class="SubPnl" method="Insert VI"(reference=w1, "VI Ref"=w7) -> ()  [unwired: 2 in, 4 out]
  n179 = invoke class="VI" method="Run VI"(reference=w28, "Wait until done"=FALSE ("Wait Until Done")) -> ()  [unwired: 3 in, 5 out]
  n180 = invoke class="VI" method="Run VI"(reference=w21, "Wait until done"=FALSE ("Wait Until Done")) -> ()  [unwired: 3 in, 5 out]
  n181 = invoke class="VI" method="Run VI"(reference=w7, "Wait until done"=FALSE ("Wait Until Done")) -> ()  [unwired: 3 in, 5 out]
